vi "GraphViz Generator UI Wrapper.vi"(10 "Modules Configurations":refnum<class "TBM module configuration.lvclass">[](array[class]), 11 "engine configuration in":refnum<class "engine configuration.lvclass">) -> ()   [LabVIEW 2013]
uses:
  <vilib>/NI/Module Execution Interface/Engine Configuration/engine configuration.lvclass
  <vilib>/NI/Tag Bus Module Framework/module configuration/TBM module configuration.lvclass
  System.Windows.Forms
  System.Drawing
  <vilib>/NI/Tag Bus Data Framework/Configuration Editor/Classes/Engine Mappings/Engine Mappings.lvclass
panel:
  in  "Tab Control":enum32{"Setup", "Image"}(tab)
  in  "Modules to View":T1(array[cluster])
  in  "Supported Colors":string[](array[string])=["dodgerblue", "cadetblue1", "darkgoldenrod1", "gainsboro", "palegreen", "peachpuff", "violet", "skyblue", "yellow", "seagreen1", "tomato", "thistle", "slateblue1", "orange", "palevioletred1"]
  in  "GraphViz 'bin' Directory":path=path "C:/Program Files (x86)/Graphviz2.38/bin"
  in  "Show Unmapped Channels?":bool=TRUE
  in  "Show Tag Labels?":bool=TRUE
  in  "Zoom?":bool=TRUE
  in  "Generate":bool
  in  "PictureBox":refnum<k24>(container)
  # "Generation Options"
  # "Supported colors list found at \nhttp://www.graphviz.org/doc/info/colors.html"
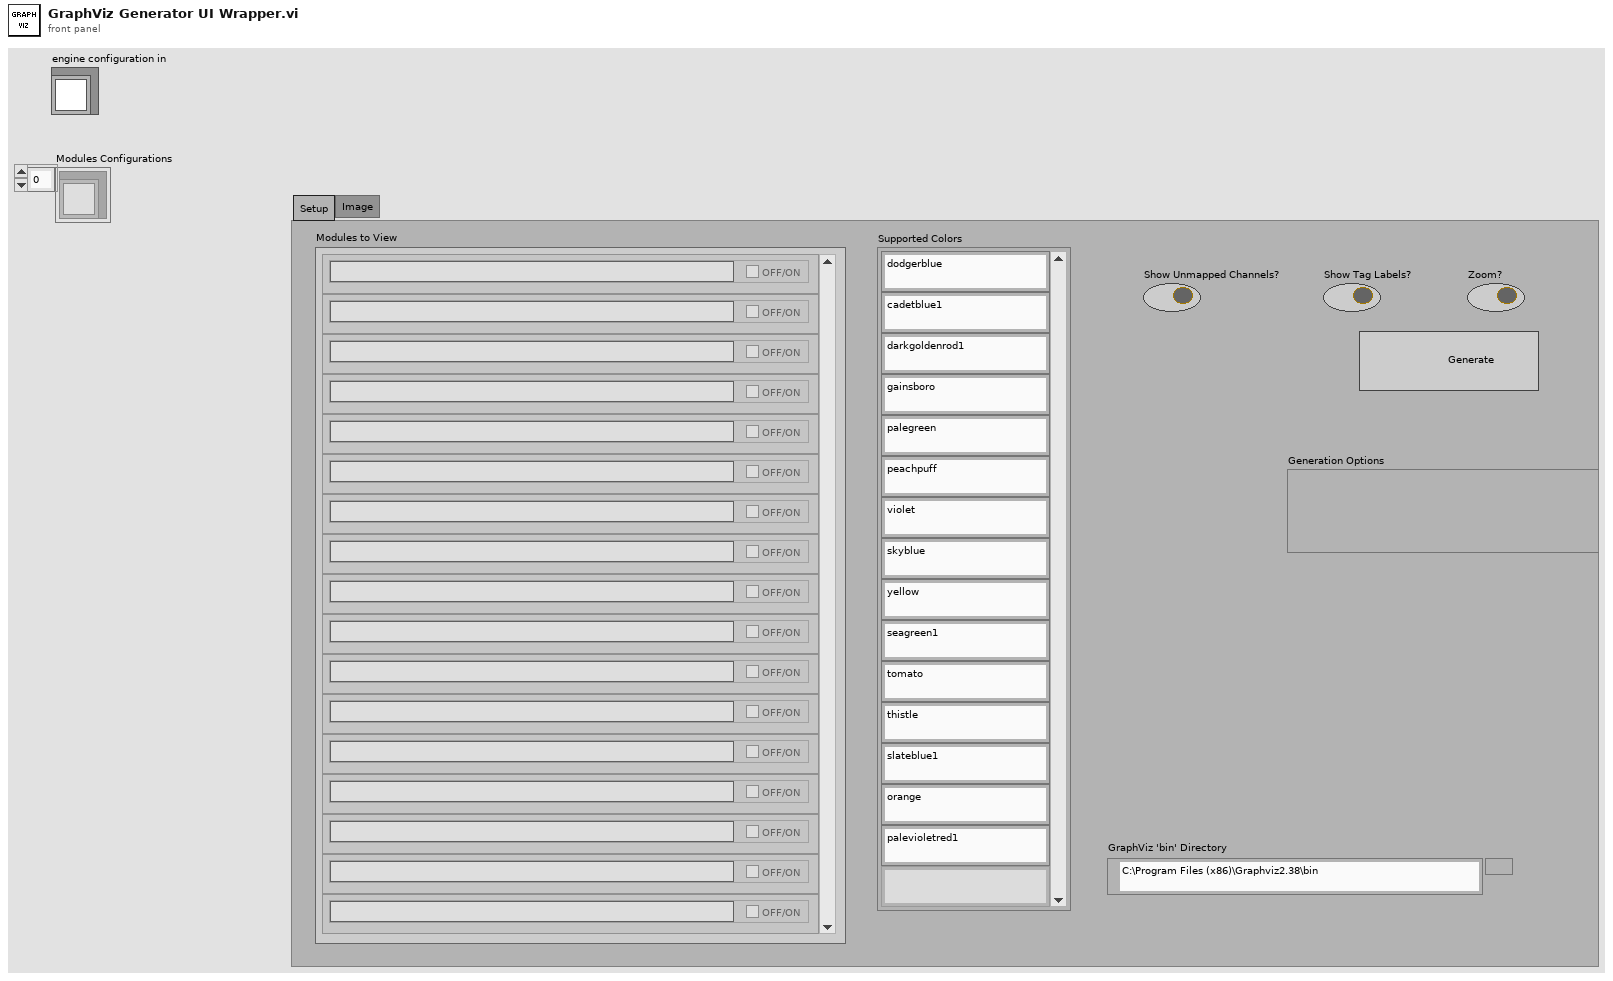
[diagram p1: front panel]
types:
  T1 = cluster{"Module Display Name":string, "View?":bool}[]
  T2 = typedef "PL Framework Configuration Tool.lvlib/Engine Mappings.lvclass/module information.ctl" = cluster{"display name":string, "instance id":string, "channels":refnum<class "TBM channel.lvclass">[]}
  T3 = cluster{"Module Display Name":string, "View?":bool}
  T4 = enum16{"open", "replace", "create", "open or create", "replace or create", "replace or create with confirmation"}
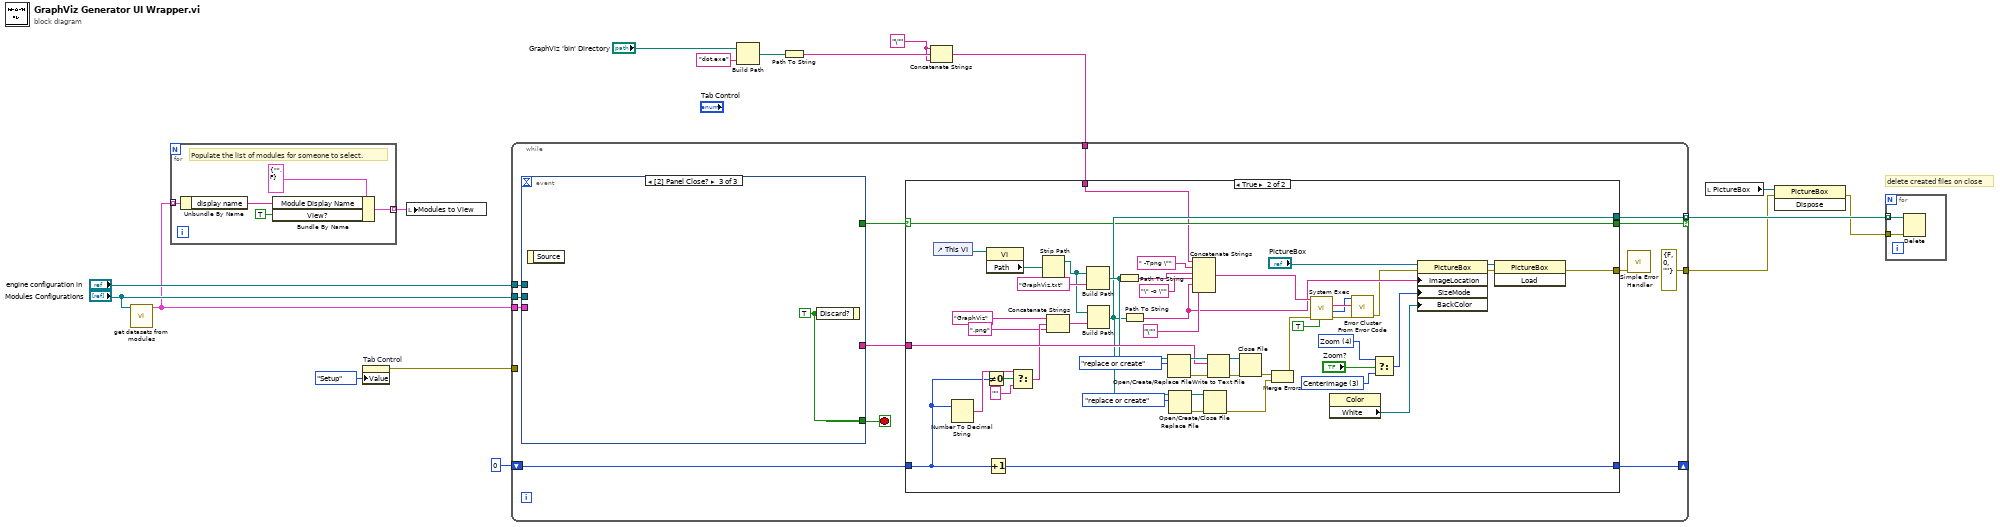
[diagram p0: block diagram]
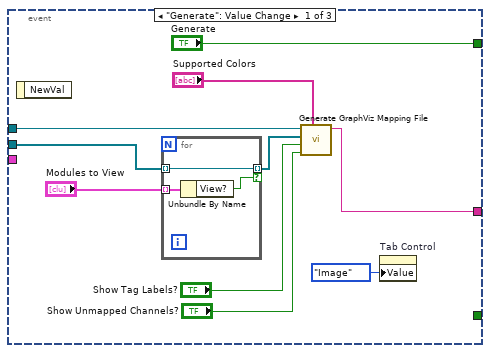
[diagram p3: hidden frame]
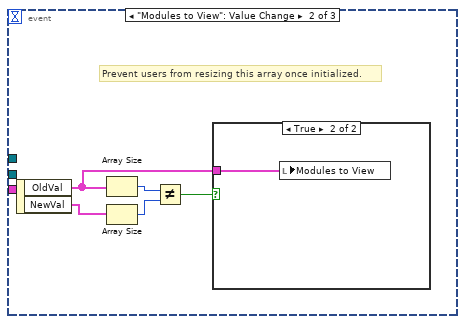
[diagram p4: hidden frame]
diagram:
  w3 = "\"" ("string")
  # "delete created files on close"
  n1 = call <vilib>:"get datasets from modules.vi"("Modules Configurations"="Modules Configurations") -> ("module datasets"=w13:T2[])  [unwired: 9 in, 1 out]
  n2 = for {
    tunnel: w13 -> [w22] mode=indexing
    tunnel: [w18] -> w12 mode=indexing
    # "Populate the list of modules for someone to select."
    n3 = Unbundle By Name(w22) -> ("display name"=w19:string)
    n4 = Bundle By Name(cluster=T3 {"Module Display Name"="", "View?"=FALSE} ("Cluster"), "Module Display Name"=w19, "View?"=TRUE) -> (w18:T3)
  }
  n5 = property on="Tab Control" class="TabCtl (strict)"("Value"=enum32{"Setup", "Image", "Text"}."Setup" ("Tab Control")) -> (error out=w1:errorcluster)  [unwired: 2 in, 1 out]
  n6 = local write "Modules to View"(w12) -> ()
  n7 = Build Path(base path="GraphViz 'bin' Directory", name or relative path="dot.exe") -> (appended path=w6:path)
  n8 = Path To String(path=w6) -> (string=w7:string)
  n9 = Concatenate Strings(w3, w7, w3) -> (w4:string)
  n10 = while {
    tunnel: "engine configuration in" -> [w35]
    tunnel: "Modules Configurations" -> [w34]
    shift-right: [w30] -> _
    shift-left: 0 -> [w29]
    tunnel: [w28] -> w15 mode=indexing if=w27
    tunnel: w13 -> [w26]
    tunnel: [errorcluster {"status"=FALSE, "code"=0, "source"=""} ("error out")] -> w10
    tunnel: w4 -> [w23]
    tunnel: w1 -> [_]
    stop <- w33 stop-if-true
    n11 = event shown="[2] Panel Close?" {
      selector: _ -> [_ _ _]
      dyn-events: _ -> [_ _ _]
      timeout: _ -> [_ _ _]
      tunnel: w35 -> [w90 _ _]
      tunnel: w34 -> [w89 _ _]
      tunnel: [_ _ w105] -> w33
      tunnel: ["Generate" _ _] -> w32
      tunnel: [w91 _ _] -> w31
      tunnel: w26 -> [_ _ _]
      event "Generate": Value Change {
        n12 = event-data() -> ()  [unwired: 1 in, 1 out]
        n13 = for {
          tunnel: "Modules to View" -> [w98] mode=indexing
          tunnel: w89 -> [w97] mode=indexing
          tunnel: [w97] -> w88 mode=indexing if=w96
          n14 = Unbundle By Name(w98) -> ("View?"=w96:bool)
        }
        n15 = call "Generate GraphViz Mapping File.vi"("supported colors"="Supported Colors", "Show Unmapped Channels?"="Show Unmapped Channels?", "Show Tag Labels?"="Show Tag Labels?", "Modules Configurations"=w88, "engine configuration in"=w90) -> ("output to graphviz"=w91:string)  [unwired: 6 in]
        n16 = property on="Tab Control" class="TabCtl (strict)"("Value"=enum32{"Setup", "Image", "Text"}."Image" ("Tab Control")) -> ()  [unwired: 2 in, 2 out]
      }
      event "Modules to View": Value Change {
        # "Prevent users from resizing this array once initialized."
        n17 = event-data() -> ("OldVal"=w99:T1, "NewVal"=w103:T1)  [unwired: 1 in]
        n18 = Array Size(array=w99) -> (size(s)=w102:i32)
        n19 = Array Size(array=w103) -> (size(s)=w101:i32)
        n20 = Not Equal?(x=w102, y=w101) -> (x != y?=w100:bool)
        n21 = case shown="True" w100 {
          tunnel: w99 -> [_ w104]
          frame False {
          }
          frame True {
            n22 = local write "Modules to View"(w104) -> ()
          }
        }
      }
      event Panel Close? {
        w105 = TRUE ("Discard?")
        n23 = event-data() -> ()  [unwired: 1 in, 1 out]
        n24 = event-data("Discard?"=w105) -> ()  [unwired: 1 in, 1 out]
      }
    }
    n25 = case shown="True" w32 {
      selector: w32 -> [_ w44]
      tunnel: w31 -> [_ w73]
      tunnel: w29 -> [w36 w52]
      tunnel: [w36 w51] -> w30
      tunnel: [_ w45] -> w28
      tunnel: [_ w44] -> w27
      tunnel: [_ w42] -> w25
      tunnel: w23 -> [_ w37]
      frame False {
      }
      frame True {
        w49 = 4 items=["Normal", "StretchImage", "AutoSize", "CenterImage", "Zoom"] ("SizeMode")
        w48 = 3 items=["Normal", "StretchImage", "AutoSize", "CenterImage", "Zoom"] ("SizeMode")
        n26 = control-ref of="This VI"() -> (w79:refnum<vi>)
        n27 = Number To Decimal String(number=w52) -> (decimal integer string=w59:string)  [unwired: 1 in]
        n28 = Not Equal To 0?(x=w52) -> (x != 0?=w60:bool)
        n29 = property class="VI"(reference=w79) -> ("Path"=w80:path)  [unwired: 1 in, 2 out]
        n30 = Increment(x=w52) -> (x+1=w51:i32)
        n31 = Select(t=w59, s=w60, f="") -> (s? t:f=w56:string)
        n32 = Strip Path(path=w80) -> (stripped path=w46:path)  [unwired: 1 out]
        n33 = Concatenate Strings("GraphViz" ("name or relative path"), w56, ".png" ("string")) -> (w54:string)
        n34 = Build Path(base path=w46, name or relative path="GraphViz.txt") -> (appended path=w67:path)
        n35 = Build Path(base path=w46, name or relative path=w54) -> (appended path=w45:path)
        n36 = Path To String(path=w67) -> (string=w82:string)
        n37 = Path To String(path=w45) -> (string=w62:string)
        n38 = Open/Create/Replace File(file path (use dialog)=w67, operation (0:open)=T4."replace or create") -> (refnum out=w74:refnum<file>, error out=w72:errorcluster)  [unwired: 4 in, 1 out]
        n39 = Open/Create/Replace File(file path (use dialog)=w45, operation (0:open)=T4."replace or create") -> (refnum out=w75:refnum<file>, error out=w76:errorcluster)  [unwired: 4 in, 1 out]
        n40 = Concatenate Strings(w37, " -Tpng \"" ("string"), w82, "\" -o \"" ("string"), w62, "\"" ("string")) -> (w66:string)
        n41 = Close File(refnum=w75, error in=w76) -> (error out=w68:errorcluster)  [unwired: 1 out]
        n42 = Write to Text File(file (use dialog)=w74, text=w73, error in=w72) -> (refnum out=w70:refnum<file>, error out=w71:errorcluster)  [unwired: 1 in, 1 out]
        n43 = Close File(refnum=w70, error in=w71) -> (error out=w69:errorcluster)  [unwired: 1 out]
        n44 = Merge Errors(w69, w68) -> (w65:errorcluster)
        n45 = call <vilib>:"System Exec.vi"("run minimized? (F)"=TRUE, "error in (no error)"=w65, "command line"=w66) -> ("error out"=w41:errorcluster, "return code"=w39:i32, "standard error"=w40:string)  [unwired: 5 in, 1 out]
        n46 = property class="Color"() -> ("White"=w53:refnum<k24>)  [unwired: 2 in, 2 out]
        n47 = call <vilib>:"Error Cluster From Error Code.vi"("error in (no error)"=w41, "error message (\"\")"=w40, "error code (0)"=w39) -> ("error out"=w38:errorcluster)  [unwired: 6 in]
        n48 = Select(t=w49, s="Zoom?", f=w48) -> (s? t:f=w47:i32)
        n49 = property class="PictureBox"(reference="PictureBox", error in=w38, "ImageLocation"=w62, "SizeMode"=w47, "BackColor"=w53) -> (reference out=w63:refnum<k24>, error out=w61:errorcluster)
        n50 = invoke class="PictureBox" method="Load"(reference=w63, error in=w61) -> (error out=w42:errorcluster)  [unwired: 1 in, 2 out]
      }
    }
    n51 = call <vilib>:"Simple Error Handler.vi"("error in (no error)"=w25) -> ()  [unwired: 4 in, 5 out]
  }
  n52 = local read "PictureBox"() -> (w11:refnum<k24>)
  n53 = invoke class="PictureBox" method="Dispose"(reference=w11, error in=w10) -> (error out=w9:errorcluster)  [unwired: 1 in, 2 out]
  n54 = for {
    tunnel: w15 -> [w107] mode=indexing
    tunnel: w9 -> [w106]
    n55 = Delete(path (use dialog)=w107, error in=w106) -> ()  [unwired: 3 in, 3 out]
  }
